vi "UI_Render.vi"(0 "Context":T1={"Screen"=enum."Settings", "Settings"=[0, 0, 1, 1], "Board"={"Grid"=array15x15[225 elements], "Move History"=[], "Last Move"={"Row"=-1, "Col"=-1, "Stone"=enum."Empty"}}, "Status"=enum."Idle", "Game ID"=0, "Player Stone"=enum."Black", "Hover"={"Row"=-1, "Col"=-1, "Stone"=enum."Empty"}, "Hover Button"=-1, "Win Line"=[], "Score 1"=0, "Score 2"=0, "Draws"=0, "Status Text"="", "Status Color"=0}, 11 "error in":errorcluster) -> (4 "Picture":picture, 15 "error out":errorcluster)   [LabVIEW 2026]
doc: "게임 Context를 화면 전체(592x780) Picture로 그린다.\n설정 화면: 갈색 배경 + 흰 카드 + 모드/선공/난이도/규칙 선택 + 게임 시작.\n게임 화면: 오목판 + 상태 카드(차례 돌, 상태, 점수) + 무르기/새 게임/설정 버튼."
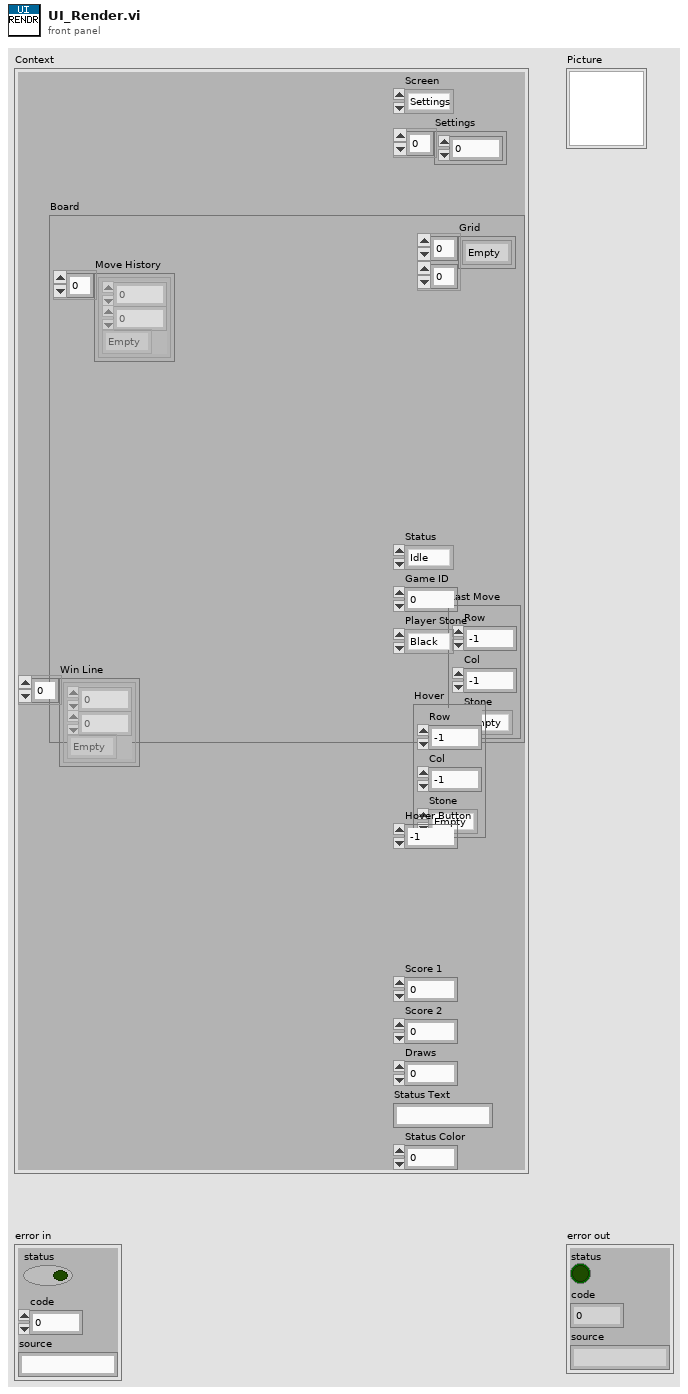
[diagram p1: front panel]
types:
  T1 = cluster{"Screen":enum16{"Settings", "Game"}, "Settings":i32[], "Board":cluster{"Grid":enum8{"Empty", "Black", "White"}[][], "Move History":cluster{"Row":i32, "Col":i32, "Stone":enum8{"Empty", "Black", "White"}}[], "Last Move":cluster{"Row":i32, "Col":i32, "Stone":enum8{"Empty", "Black", "White"}}}, "Status":enum16{"Idle", "Player Turn", "AI Thinking", "Game Over"}, "Game ID":u32, "Player Stone":enum8{"Empty", "Black", "White"}, "Hover":cluster{"Row":i32, "Col":i32, "Stone":enum8{"Empty", "Black", "White"}}, "Hover Button":i32, "Win Line":cluster{"Row":i32, "Col":i32, "Stone":enum8{"Empty", "Black", "White"}}[], "Score 1":i32, "Score 2":i32, "Draws":i32, "Status Text":string, "Status Color":u32}
  T2 = cluster{"Font Name:":string, "Size":i16, "Strikeout?":bool, "Italic?":bool, "Underline?":bool, "Outline?":bool, "Shadow?":bool, "Bold?":bool}
  T3 = enum16{"User-specified Font", "Application Font", "System Font", "Dialog Font"}
  T4 = cluster{"horizontal":enum16{"left", "center", "right"}, "vertical":enum16{"top", "center", "bottom"}}
  T5 = enum16{"Idle", "Player Turn", "AI Thinking", "Game Over"}
  T6 = cluster{"left":i16, "top":i16, "right":i16, "bottom":i16}
  T7 = cluster{"Grid":enum8{"Empty", "Black", "White"}[][], "Move History":cluster{"Row":i32, "Col":i32, "Stone":enum8{"Empty", "Black", "White"}}[], "Last Move":cluster{"Row":i32, "Col":i32, "Stone":enum8{"Empty", "Black", "White"}}}
  T8 = cluster{"Row":i32, "Col":i32, "Stone":enum8{"Empty", "Black", "White"}}
  T9 = cluster{"Row":i32, "Col":i32, "Stone":enum8{"Empty", "Black", "White"}}[]
  T10 = cluster{"Rect":cluster{"left":i16, "top":i16, "right":i16, "bottom":i16}, "Fill":u32, "Fill Sel":u32, "Border":u32, "Border Sel":u32, "Text":string, "Text Color":u32, "Text Sel":u32, "Size":i16, "Bold":bool, "Group":i32, "Value":i32, "Radius":i16}[]
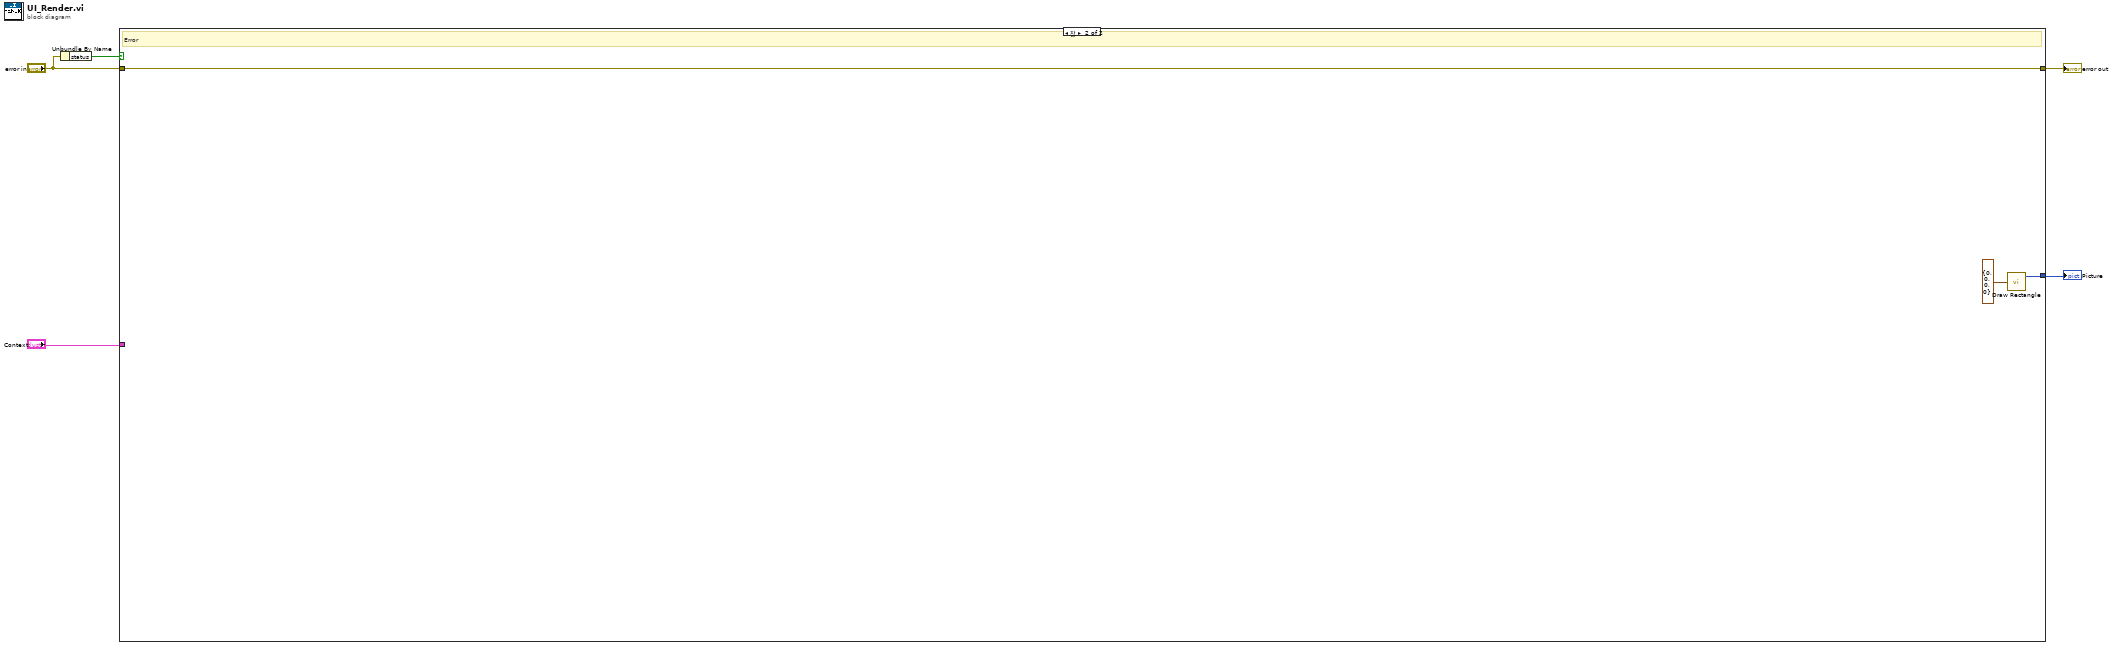
[diagram p0: block diagram]
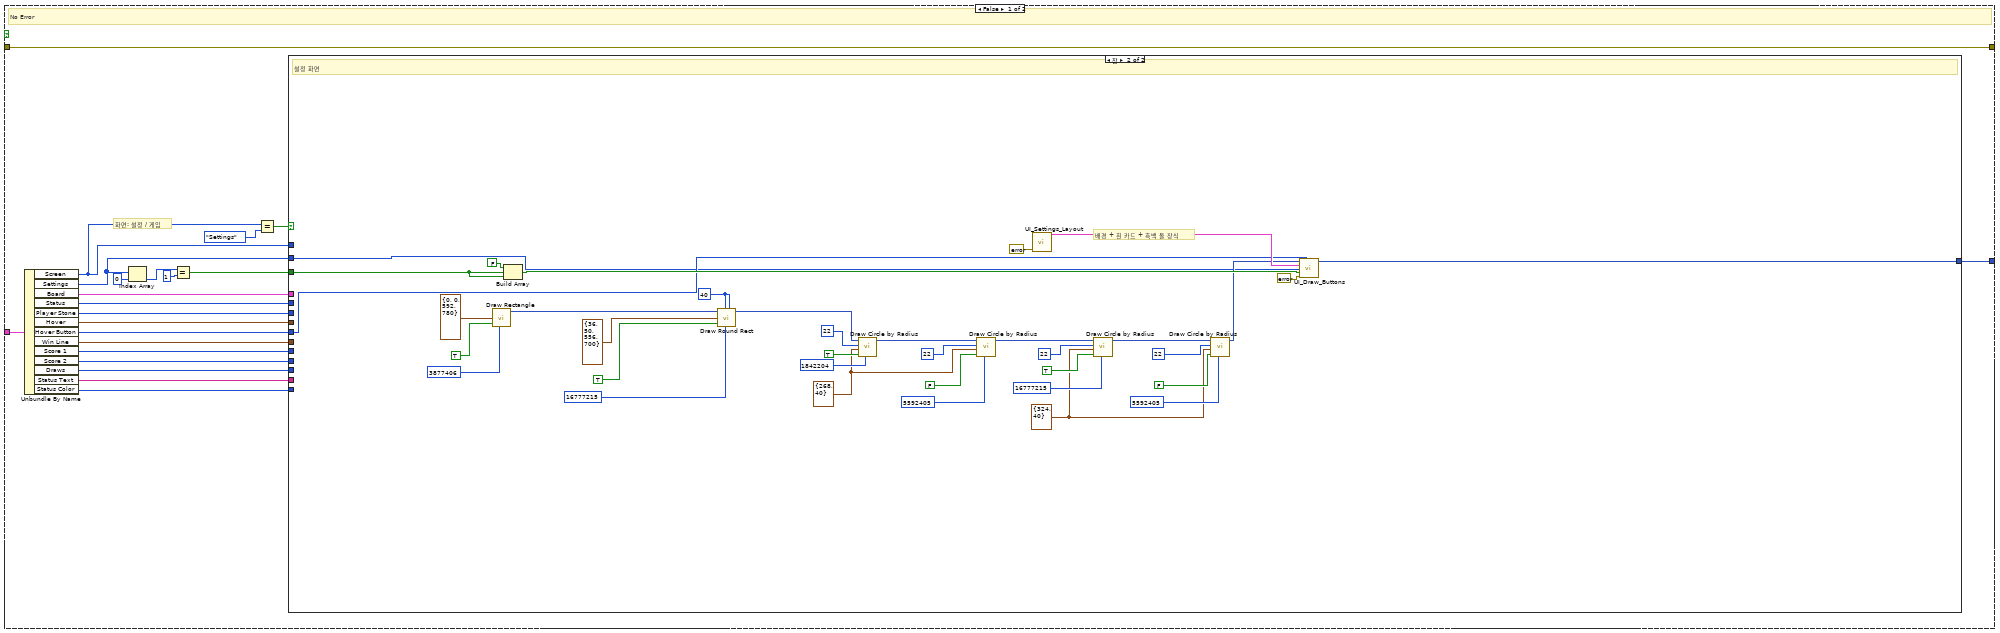
[diagram p2: hidden frame]
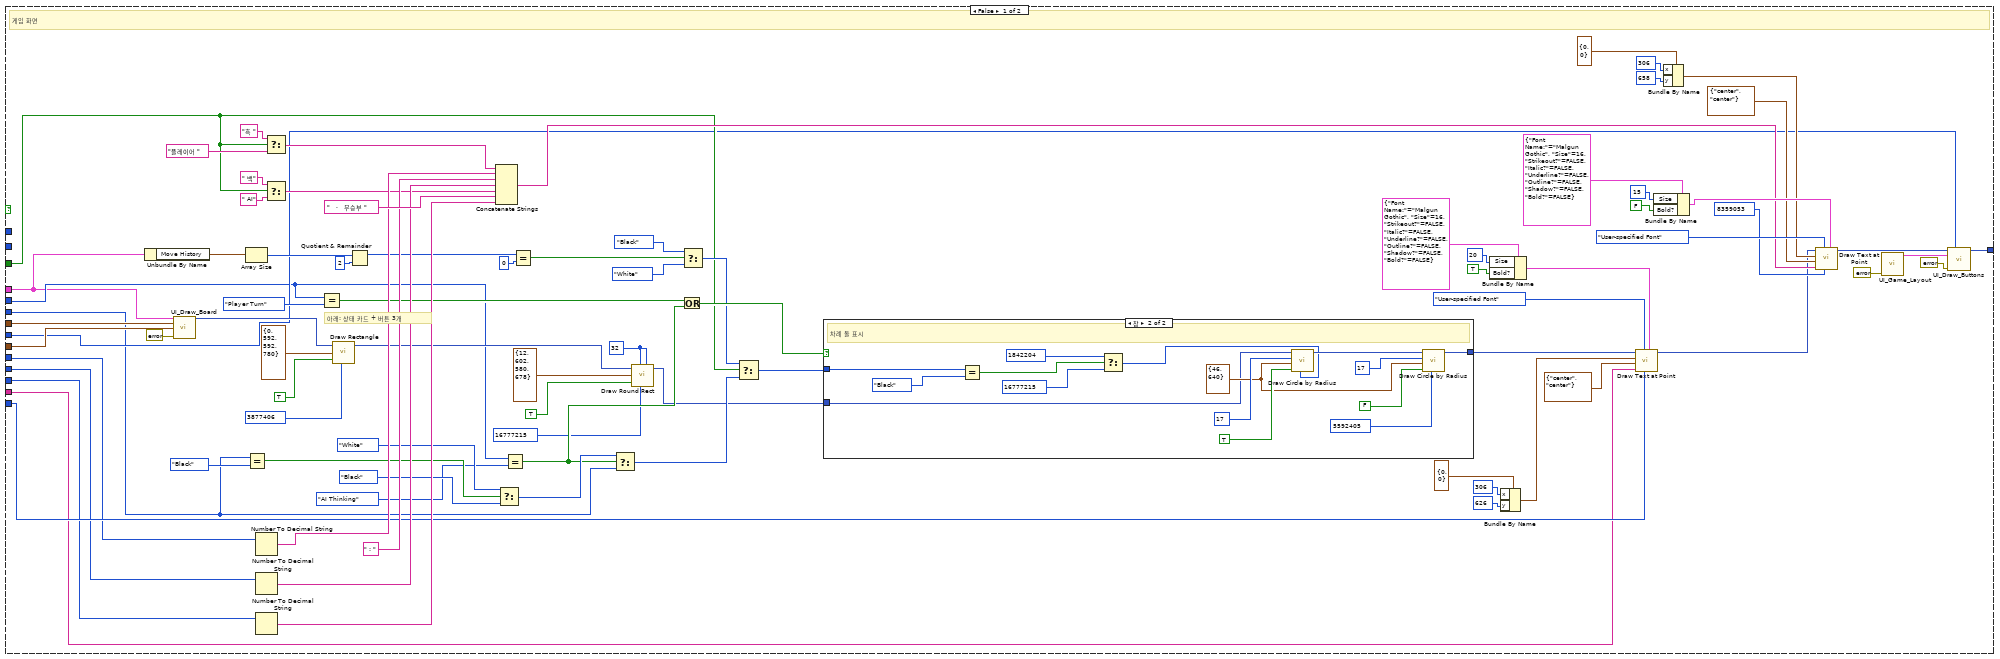
[diagram p3: hidden frame]
diagram:
  n1 = Unbundle By Name("error in") -> ("status"=w3:bool)
  n2 = case shown="참" w3 {
    tunnel: "Context" -> [w6 _]
    tunnel: "error in" -> [w7 w164]
    tunnel: [w7 w164] -> w5
    tunnel: [w27 w166] -> w4
    frame False {
      # "화면: 설정 / 게임"
      # "No Error"
      n3 = Unbundle By Name(w6) -> ("Screen"=w8:enum16{"Settings", "Game"}, "Settings"=w9:i32[], "Board"=w10:T7, "Status"=w11:T5, "Player Stone"=w12:enum8{"Empty", "Black", "White"}, "Hover"=w13:T8, "Hover Button"=w14:i32, "Win Line"=w15:T9, "Score 1"=w16:i32, "Score 2"=w17:i32, "Draws"=w18:i32, "Status Text"=w19:string, "Status Color"=w20:u32)
      n4 = Index Array(array=w9, index=0) -> (element=w22:i32)
      n5 = Equal?(x=w22, y=1) -> (x = y?=w24:bool)
      n6 = Equal?(x=w8, y=enum16{"Settings", "Game"}."Settings") -> (x = y?=w26:bool)
      n7 = case shown="참" w26 {
        tunnel: w8 -> [_ _]
        tunnel: w9 -> [_ w128]
        tunnel: w10 -> [w28 _]
        tunnel: w11 -> [w29 _]
        tunnel: w12 -> [w30 _]
        tunnel: w13 -> [w31 _]
        tunnel: w14 -> [w32 w129]
        tunnel: w15 -> [w33 _]
        tunnel: w16 -> [w34 _]
        tunnel: w17 -> [w35 _]
        tunnel: w18 -> [w36 _]
        tunnel: w19 -> [w37 _]
        tunnel: w20 -> [w38 _]
        tunnel: w24 -> [w39 w130]
        tunnel: [w111 w163] -> w27
        frame False {
          w48 = i16 32
          # "아래: 상태 카드 + 버튼 3개"
          # "게임 화면"
          n8 = Unbundle By Name(w28) -> ("Move History"=w51:T9)
          n9 = call "UI_Draw_Board.vi"("Board State"=w28, "Hover"=w31, "Win Line"=w33, "error in"=errorcluster {"status"=FALSE, "code"=0, "source"=""}) -> ("Picture"=w41:picture)  [unwired: 10 in, 1 out]
          n10 = Array Size(array=w51) -> (size(s)=w52:i32)
          n11 = Equal?(x=w30, y=enum8{"Empty", "Black", "White"}."Black") -> (x = y?=w63:bool)
          n12 = Number To Decimal String(number=w34) -> (decimal integer string=w90:string)  [unwired: 1 in]
          n13 = Number To Decimal String(number=w35) -> (decimal integer string=w92:string)  [unwired: 1 in]
          n14 = Number To Decimal String(number=w36) -> (decimal integer string=w94:string)  [unwired: 1 in]
          n15 = Select(t="흑 ", s=w39, f="플레이어 ") -> (s? t:f=w86:string)
          n16 = Select(t=" 백", s=w39, f=" AI") -> (s? t:f=w89:string)
          n17 = Equal?(x=w29, y=T5."Player Turn") -> (x = y?=w70:bool)
          n18 = call <vilib>:"Draw Rectangle.vi"("picture"=w41, "rect"=T6 {"left"=0, "top"=592, "right"=592, "bottom"=780}, "fill?(F)"=TRUE, "color(black)"=u32 3877406) -> ("new picture"=w45:picture)  [unwired: 5 in]
          n19 = Quotient & Remainder(x=w52, y=2) -> (x-y*floor(x/y)=w54:i32)  [unwired: 1 out]
          n20 = Concatenate Strings(w86, w90, " : ", w92, w89, "   ·   무승부 ", w94) -> (w95:string)
          n21 = Select(t=enum8{"Empty", "Black", "White"}."White", s=w63, f=enum8{"Empty", "Black", "White"}."Black") -> (s? t:f=w66:enum8{"Empty", "Black", "White"})
          n22 = Equal?(x=w29, y=T5."AI Thinking") -> (x = y?=w61:bool)
          n23 = Equal?(x=w54, y=0) -> (x = y?=w58:bool)
          n24 = Select(t=w66, s=w61, f=w30) -> (s? t:f=w67:enum8{"Empty", "Black", "White"})
          n25 = call <vilib>:"Draw Round Rect.vi"("picture"=w45, "oval width"=w48, "rect"=T6 {"left"=12, "top"=602, "right"=580, "bottom"=678}, "fill?(F)"=TRUE, "color(black)"=u32 16777215, "oval height"=w48) -> ("new picture"=w50:picture)  [unwired: 3 in]
          n26 = Or(x=w70, y=w61) -> (x .or. y?=w71:bool)
          n27 = Select(t=enum8{"Empty", "Black", "White"}."Black", s=w58, f=enum8{"Empty", "Black", "White"}."White") -> (s? t:f=w59:enum8{"Empty", "Black", "White"})
          n28 = Select(t=w59, s=w39, f=w67) -> (s? t:f=w68:enum8{"Empty", "Black", "White"})
          n29 = case shown="참" w71 {
            tunnel: w50 -> [w112 w113]
            tunnel: w68 -> [_ w114]
            tunnel: [w112 w127] -> w72
            frame False {
              # "표시 안 함"
            }
            frame True {
              w120 = cluster{"horizontal":i16, "vertical":i16} {"horizontal"=46, "vertical"=640}
              # "차례 돌 표시"
              n30 = Equal?(x=w114, y=enum8{"Empty", "Black", "White"}."Black") -> (x = y?=w116:bool)
              n31 = Select(t=u32 1842204, s=w116, f=u32 16777215) -> (s? t:f=w119:u32)
              n32 = call <vilib>:"Draw Circle by Radius.vi"("color(black)"=w119, "fill?(F)"=TRUE, "pixel center"=w120, "radius"=i16 17, "picture"=w113) -> ("new picture"=w123:picture)  [unwired: 6 in]
              n33 = call <vilib>:"Draw Circle by Radius.vi"("color(black)"=u32 5592405, "fill?(F)"=FALSE, "pixel center"=w120, "radius"=i16 17, "picture"=w123) -> ("new picture"=w127:picture)  [unwired: 6 in]
            }
          }
          n34 = Bundle By Name(cluster=T2 {"Font Name:"="Malgun Gothic", "Size"=16, "Strikeout?"=FALSE, "Italic?"=FALSE, "Underline?"=FALSE, "Outline?"=FALSE, "Shadow?"=FALSE, "Bold?"=FALSE}, "Size"=i16 20, "Bold?"=TRUE) -> (w82:T2)
          n35 = Bundle By Name(cluster=cluster{"x":i16, "y":i16} {"x"=0, "y"=0}, "x"=i16 306, "y"=i16 626) -> (w78:cluster{"x":i16, "y":i16})
          n36 = call <vilib>:"Draw Text at Point.vi"("[user-specified font]"=w82, "text color(black)"=w38, "desired font(Application)"=T3."User-specified Font", "text"=w37, "alignment(left, top)"=T4 {"horizontal"=enum."center", "vertical"=enum."center"}, "origin"=w78, "picture"=w72) -> ("new picture"=w83:picture)  [unwired: 3 in, 1 out]
          n37 = Bundle By Name(cluster=T2 {"Font Name:"="Malgun Gothic", "Size"=16, "Strikeout?"=FALSE, "Italic?"=FALSE, "Underline?"=FALSE, "Outline?"=FALSE, "Shadow?"=FALSE, "Bold?"=FALSE}, "Size"=i16 15, "Bold?"=FALSE) -> (w106:T2)
          n38 = Bundle By Name(cluster=cluster{"x":i16, "y":i16} {"x"=0, "y"=0}, "x"=i16 306, "y"=i16 658) -> (w102:cluster{"x":i16, "y":i16})
          n39 = call <vilib>:"Draw Text at Point.vi"("[user-specified font]"=w106, "text color(black)"=u32 8359053, "desired font(Application)"=T3."User-specified Font", "text"=w95, "alignment(left, top)"=T4 {"horizontal"=enum."center", "vertical"=enum."center"}, "origin"=w102, "picture"=w83) -> ("new picture"=w107:picture)  [unwired: 3 in, 1 out]
          n40 = call "UI_Game_Layout.vi"("error in"=errorcluster {"status"=FALSE, "code"=0, "source"=""}) -> ("Specs"=w109:T10)  [unwired: 13 in, 1 out]
          n41 = call "UI_Draw_Buttons.vi"("Picture"=w107, "Hover"=w32, "Specs"=w109, "error in"=errorcluster {"status"=FALSE, "code"=0, "source"=""}) -> ("New Picture"=w111:picture)  [unwired: 10 in, 1 out]
        }
        frame True {
          w149 = cluster{"horizontal":i16, "vertical":i16} {"horizontal"=324, "vertical"=40}
          w140 = cluster{"horizontal":i16, "vertical":i16} {"horizontal"=268, "vertical"=40}
          w137 = i16 40
          # "배경 + 흰 카드 + 흑백 돌 장식"
          # "설정 화면"
          n42 = call <vilib>:"Draw Rectangle.vi"("rect"=T6 {"left"=0, "top"=0, "right"=592, "bottom"=780}, "fill?(F)"=TRUE, "color(black)"=u32 3877406) -> ("new picture"=w134:picture)  [unwired: 6 in]
          n43 = Build Array(FALSE, w130, w130) -> (w161:bool[])
          n44 = call <vilib>:"Draw Round Rect.vi"("picture"=w134, "oval width"=w137, "rect"=T6 {"left"=36, "top"=50, "right"=556, "bottom"=700}, "fill?(F)"=TRUE, "color(black)"=u32 16777215, "oval height"=w137) -> ("new picture"=w139:picture)  [unwired: 3 in]
          n45 = call <vilib>:"Draw Circle by Radius.vi"("color(black)"=u32 1842204, "fill?(F)"=TRUE, "pixel center"=w140, "radius"=i16 22, "picture"=w139) -> ("new picture"=w144:picture)  [unwired: 6 in]
          n46 = call <vilib>:"Draw Circle by Radius.vi"("color(black)"=u32 5592405, "fill?(F)"=FALSE, "pixel center"=w140, "radius"=i16 22, "picture"=w144) -> ("new picture"=w148:picture)  [unwired: 6 in]
          n47 = call "UI_Settings_Layout.vi"("error in"=errorcluster {"status"=FALSE, "code"=0, "source"=""}) -> ("Specs"=w159:T10)  [unwired: 13 in, 1 out]
          n48 = call <vilib>:"Draw Circle by Radius.vi"("color(black)"=u32 16777215, "fill?(F)"=TRUE, "pixel center"=w149, "radius"=i16 22, "picture"=w148) -> ("new picture"=w153:picture)  [unwired: 6 in]
          n49 = call <vilib>:"Draw Circle by Radius.vi"("color(black)"=u32 5592405, "fill?(F)"=FALSE, "pixel center"=w149, "radius"=i16 22, "picture"=w153) -> ("new picture"=w157:picture)  [unwired: 6 in]
          n50 = call "UI_Draw_Buttons.vi"("Picture"=w157, "Hover"=w129, "Specs"=w159, "Values"=w128, "Dim Groups"=w161, "error in"=errorcluster {"status"=FALSE, "code"=0, "source"=""}) -> ("New Picture"=w163:picture)  [unwired: 8 in, 1 out]
        }
      }
    }
    frame True {
      # "Error"
      n51 = call <vilib>:"Draw Rectangle.vi"("rect"=T6 {"left"=0, "top"=0, "right"=0, "bottom"=0}) -> ("new picture"=w166:picture)  [unwired: 8 in]
    }
  }
  "Picture" <- w4
  "error out" <- w5
